vi "DC Motor Controller (FPGA).vi"() -> ()   [LabVIEW 2017]
doc: "Implements the FPGA controller of the Robotics Starter Kit motors.\n\nThis example is configured to run on a Single-board RIO 9631 and needs to be compiled. If you have a different RIO device, you must add the appropriate RIO targets to your LabVIEW Project and move the VIs in this project to the new target. You must also configure the IP address of the RIO target to match your network configuration."
uses:
  <vilib>/Platform/TimedLoop/XDataNode/timing_clust.ctl
  <vilib>/Platform/TimedLoop/XDataNode/nitl_modes.ctl
  <vilib>/Platform/TimedLoop/XDataNode/wakeup.ctl
  <vilib>/robotics/Utilities/Encoder Count Encoding.ctl
  <vilib>/rvi/Emulation/niFpgaSctlEmulationGetInTimedLoop.vi
  <vilib>/rvi/Emulation/niFpgaProcessEmulError.vi
  <vilib>/robotics/Utilities/FPGA Utilities/Count Two Phase Digital Encoder.vi
  <vilib>/rvi/eio/common/nirviEmuTemplateMethod_errors.vi
  <vilib>/rvi/Emulation/niFpgaGetClockAttributes.vi
  <vilib>/rvi/Emulation/niFpgaEmulationReportErrorSimple.vi
  Support VIs/DCMotor FPGA Globals.vi
  <vilib>/robotics/Utilities/FPGA Utilities/Generate Digital Pulse (uSec).vi
  <vilib>/rvi/Emulation/niFpgaCriticalErrorInLSC.vi
  <vilib>/eio/EIONode/EIONode.xnode
  <vilib>/addons/control/pid/fpga.llb/XNode/niFpgaPID.xnode
  <vilib>/Platform/TimedLoop/XDataNode/XDataNode.xnode
  <vilib>/robotics/Utilities/NI_Robotics Utilities.lvlib
  <vilib>/Platform/TimedLoop/XDataNode/XDNodeRunTimeDep.lvlib
  <vilib>/robotics/Utilities/FPGA Utilities/NI_Robotics_FPGA Utilities.lvlib
panel:
  in  "S 7":bool
  in  "Servo 7":u32(slide) scale=0.0..3000.0
  in  "invert pulse (F)":bool=TRUE
  in  "S6_timer":u16
  in  "S6_prev":u32
  in  "Indication":bool
  out "M1_finished":bool
  out "M0_finished":bool
  in  "DCmotor_1_B":bool
  in  "DCmotor_0_B":bool
  in  "M2_B":bool
  in  "Motor Power":u32(slide) scale=0.0..1000.0
  in  "M2_A":bool
  in  "Servo 4":u32(slide) scale=0.0..3000.0
  in  "Servo 5":u32(slide) scale=0.0..3000.0
  in  "Servo 6":u32(slide) scale=0.0..3000.0
  in  "S 4":bool
  in  "S 5":bool
  in  "S 6":bool
  in  "Slow velocity":i32=5
  in  "Ticks to slow":i32=360
  in  "Ticks to stop":i32=6
  in  "DCmotor_1_enc trgt":i32
  in  "DCmotor_0_enc trgt":i32
  in  "Left Encoder B":refnum<k21>="ConnectorB/DIO4"
  in  "Left Encoder A":refnum<k21>="ConnectorB/DIO3"
  in  "Right Encoder B":refnum<k21>="ConnectorA/DIO4"
  in  "Right Encoder A":refnum<k21>="ConnectorA/DIO3"
  in  "Right Motor":refnum<k21>="ConnectorB/DIO9"
  in  "Left Motor":refnum<k21>="ConnectorB/DIO8"
  in  "M0_B":refnum<k21>="ConnectorB/DIO6"
  in  "M0_A":refnum<k21>="ConnectorB/DIO5"
  in  "M1_B":refnum<k21>="ConnectorB/DIO7"
  in  "M1_A":refnum<k21>="ConnectorB/DIO13"
  out "DCmotor_0_enc":i32
  out "DCmotor_1_enc":i32
  in  "DCmotor_1_A":bool
  in  "DCmotor_0_A":bool
  in  "stop":bool
  in  "motor PID gains":T1={"proportional gain (Kc)"=2.5, "integral gain (Kc*Ts/Ti)"=0.01171875, "derivative gain (Kc*Td/Ts)"=0.01171875}
  in  "DCmotor_0_ccw vel sp":i32
  in  "DCmotor_1_ccw vel sp":i32
  out "DCmotor_0_ccw vel":i32
  out "DCmotor_1_ccw vel":i32
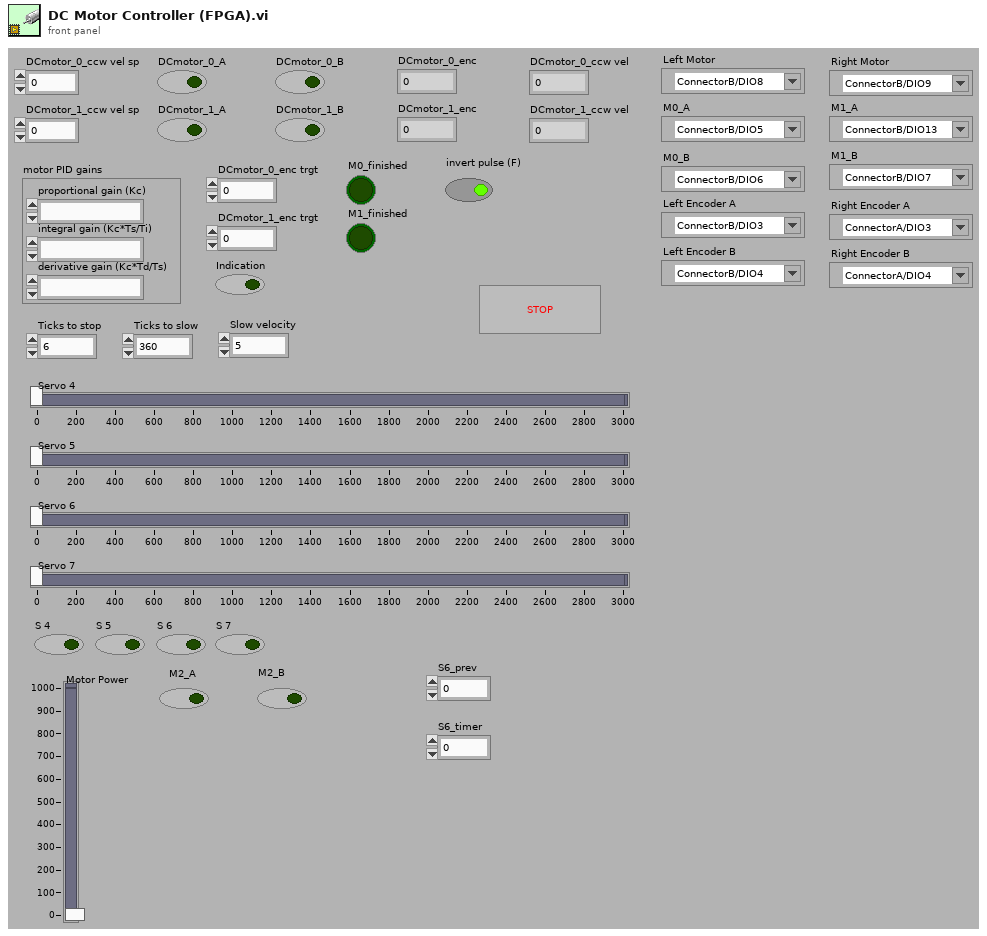
[diagram p1: front panel]
types:
  T1 = cluster{"proportional gain (Kc)":fxp<+/-,16,8>, "integral gain (Kc*Ts/Ti)":fxp<+/-,16,8>, "derivative gain (Kc*Td/Ts)":fxp<+/-,16,8>}
  T2 = cluster{"PID gains":cluster{"proportional gain (Kc)":fxp<+/-,16,8>, "integral gain (Kc*Ts/Ti)":fxp<+/-,16,8>, "derivative gain (Kc*Td/Ts)":fxp<+/-,16,8>}, "output range":cluster{"output high":fxp<+/-,16,16>, "output low":fxp<+/-,16,16>}, "setpoint":fxp<+/-,16,16>, "channel index":u16}
  T3 = cluster{"PID gains (x 2^8)":cluster{"proportional gain (Kc)":i16, "integral gain (Kc*Ts/Ti)":i16, "derivative gain (Kc*Td/Ts)":i16}, "output range":cluster{"output high":i16, "output low":i16}, "setpoint":i16, "channel index":u16}
  T4 = typedef "XDNodeRunTimeDep.lvlib/timing_clust.ctl" = cluster{"Expected End [f-1]":u64, "Actual End [f-1]":u64, "Finished Late? [f-1]":bool, "Expected End [i-1]":u64, "Actual End [i-1]":u64, "Finished Late? [i-1]":bool, "Expected Start [i]":u64, "Actual Start [i]":u64, "Expected Start [f]":u64, "Actual Start [f]":u64, "Source Name":string, "Structure Name":string, "Period":i64, "Deadline":i64, "Offset":i64, "Start":i64, "Priority":i32, "Timeout":i32, "Mode":T5, "Wakeup Reason":T6, "Error":errorcluster, "Source Type":string, "Secondary Source Type":string, "Global End Time":u64, "Global Start Time":u64, "Frame Duration":u64, "Iteration Duration":u64, "Assigned CPU":i32, "I/O Scan Engine Mode":u32}
  T5 = typedef "XDNodeRunTimeDep.lvlib/nitl_modes.ctl" = enum32{"No Change", "Process missed periods, maintain original phase", "Discard missed periods, maintain original phase", "Process missed periods, ignore original phase", "Discard missed periods, ignore original phase"}
  T6 = typedef "XDNodeRunTimeDep.lvlib/wakeup.ctl" = enum32{"Normal", "Aborted", "Asynchronous wakeup", "Timing source error", "Timed loop error", "Timeout"}
  T7 = typedef "NI_Robotics Utilities.lvlib/Encoder Count Encoding.ctl" = enum16{"X1", "X2", "X4"}
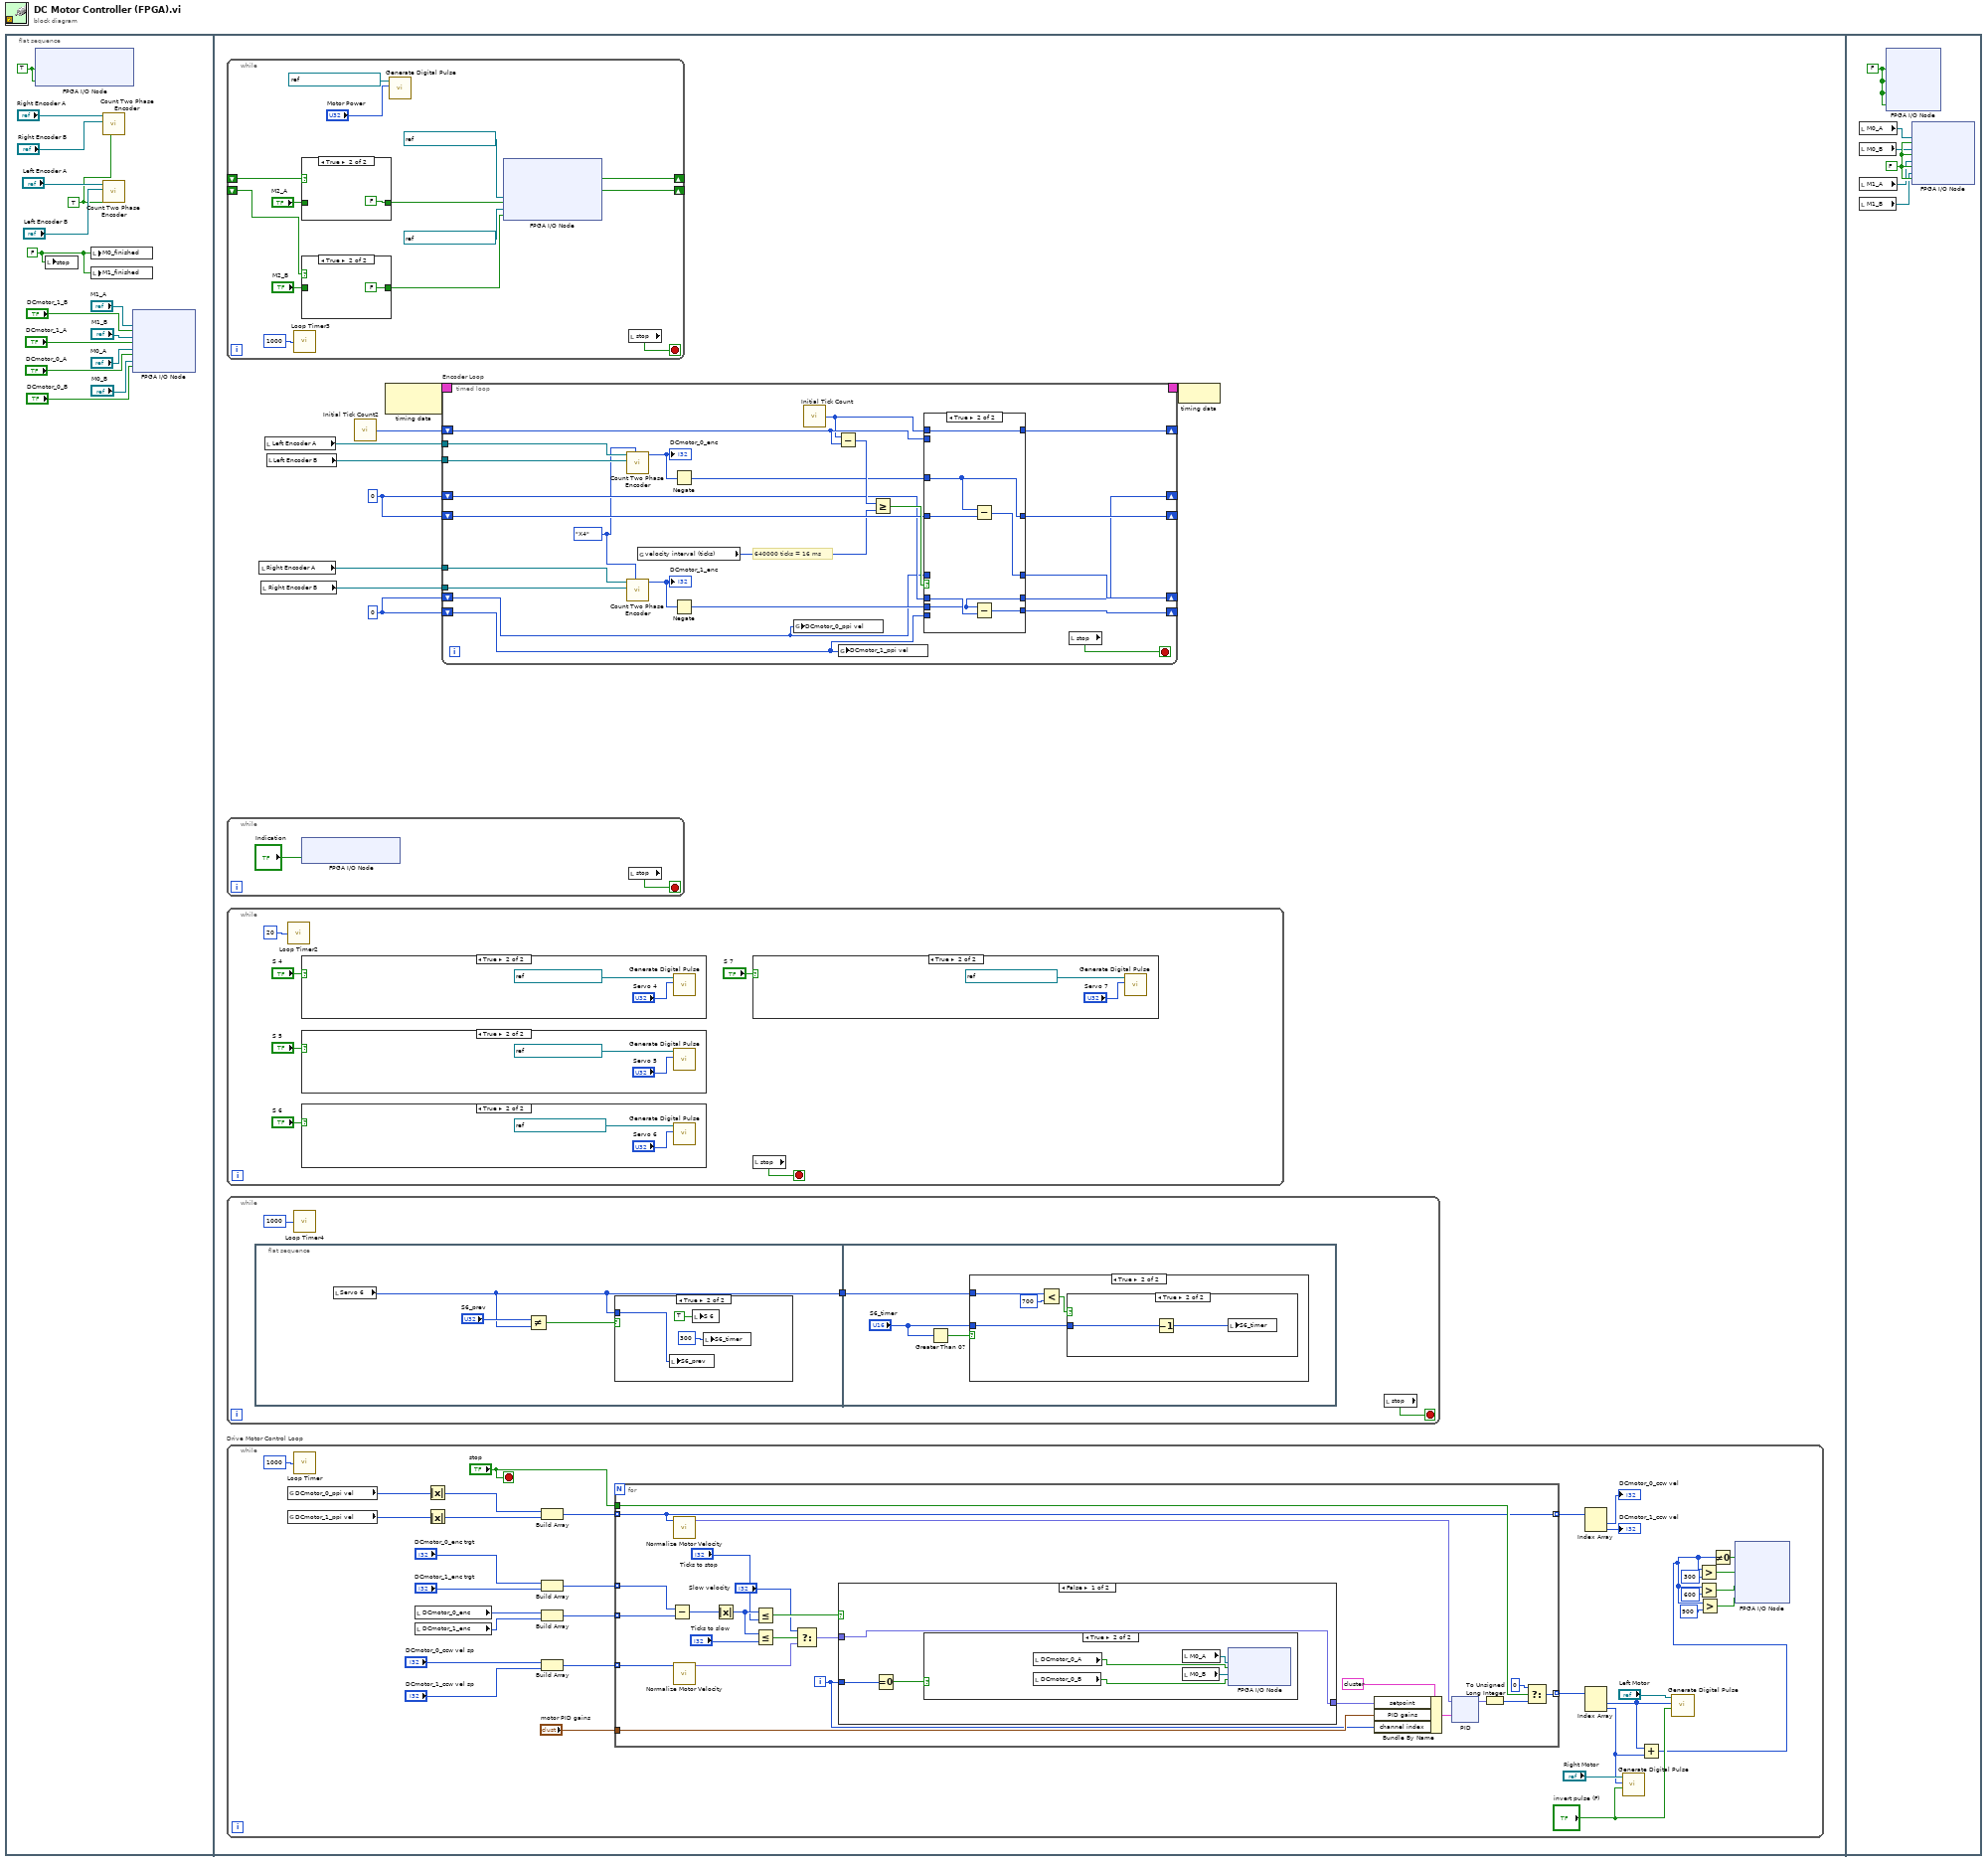
[diagram p0: block diagram]
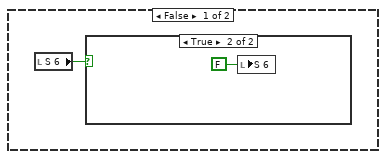
[diagram p3: hidden frame]
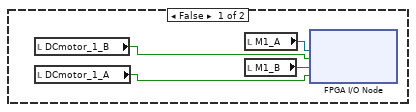
[diagram p12: hidden frame]
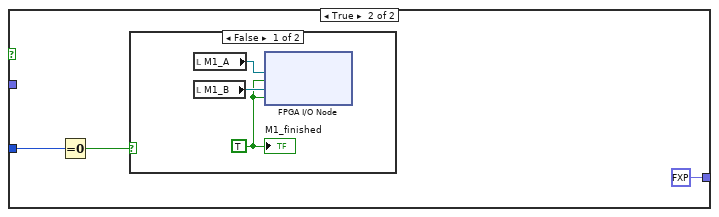
[diagram p13: hidden frame]
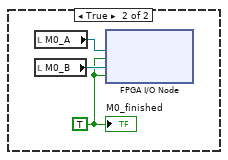
[diagram p14: hidden frame]
diagram:
  n1 = flat-sequence {
    frame #0 {
      w6 = TRUE ("ConnectorC/DIO0")
      w11 = TRUE ("reset (F)")
      w1 = FALSE ("stop")
      n2 = xnode "FPGA I/O Node"("ConnectorC/DIO2"=w6, "ConnectorC/DIO4"=w6) -> ()  [unwired: 2 in, 2 out]
      n3 = local write "stop"(w1) -> ()
      n4 = local write "M0_finished"(w1) -> ()
      n5 = local write "M1_finished"(w1) -> ()
      n6 = call-poly <vilib>:"Count Two Phase Encoder.vi"("reset (F)"=w11, "phase B FPGA digital input"="Right Encoder B", "phase A FPGA digital input"="Right Encoder A") -> ()  [unwired: 7 in, 2 out]
      n7 = call-poly <vilib>:"Count Two Phase Encoder.vi"("reset (F)"=w11, "phase B FPGA digital input"="Left Encoder B", "phase A FPGA digital input"="Left Encoder A") -> ()  [unwired: 7 in, 2 out]
      n8 = xnode "FPGA I/O Node"("I/O Item"="DCmotor_1_B", "FPGA I/O In"="M1_A", "I/O Item"="DCmotor_1_A", "FPGA I/O In"="M1_B", "I/O Item"="DCmotor_0_A", "FPGA I/O In"="M0_A", "I/O Item"="DCmotor_0_B", "FPGA I/O In"="M0_B") -> ()  [unwired: 4 out]
    }
    frame #1 {
      w20 = 0
      w21 = 0 ("Reset Position Value")
      n9 = while {
        shift-right: [w52] -> _
        shift-left: _ -> [w51]
        shift-right: [w50] -> _
        shift-left: _ -> [w49]
        stop <- w55 stop-if-true
        n10 = call "Loop Timer3"("Count(uSec)"=u32 1000) -> ()  [unwired: 1 out]
        n11 = case shown="True" w51 {
          tunnel: [w63 FALSE] -> w54
          tunnel: "M2_A" -> [w63 _]
          frame False {
          }
          frame True {
          }
        }
        n12 = case shown="True" w49 {
          tunnel: [w61 FALSE] -> w47
          tunnel: "M2_B" -> [w61 _]
          frame False {
          }
          frame True {
          }
        }
        n13 = call-poly <vilib>:"Generate Digital Pulse.vi"("pulse width (uSec)"="Motor Power", "FPGA digital output"=refnum<k21> "ConnectorA/DIO15") -> ()  [unwired: 10 in]
        n14 = xnode "FPGA I/O Node"("I/O Item"=w54, "FPGA I/O In"=refnum<k21> "ConnectorA/DIO14", "I/O Item"=w47, "FPGA I/O In"=refnum<k21> "ConnectorA/DIO13") -> ("ConnectorC/DIO1"=w52:bool, "ConnectorC/DIO3"=w50:bool)  [unwired: 2 in, 4 out]
        n15 = local read "stop"() -> (w55:bool)
      }
      n16 = while {
        stop <- w45 stop-if-true
        n17 = xnode "FPGA I/O Node"("ConnectorC/DIO0"="Indication") -> ()  [unwired: 1 in, 1 out]
        n18 = local read "stop"() -> (w45:bool)
      }
      n19 = while {
        stop <- w66 stop-if-true
        n20 = call "Loop Timer2"("Count(mSec)"=u32 20) -> ()  [unwired: 1 out]
        n21 = case shown="True" "S 4" {
          frame False {
          }
          frame True {
            n22 = call-poly <vilib>:"Generate Digital Pulse.vi"("pulse width (uSec)"="Servo 4", "FPGA digital output"=refnum<k21> "ConnectorA/DIO8") -> ()  [unwired: 10 in]
          }
        }
        n23 = case shown="True" "S 5" {
          frame False {
          }
          frame True {
            n24 = call-poly <vilib>:"Generate Digital Pulse.vi"("pulse width (uSec)"="Servo 5", "FPGA digital output"=refnum<k21> "ConnectorA/DIO9") -> ()  [unwired: 10 in]
          }
        }
        n25 = case shown="True" "S 6" {
          frame False {
          }
          frame True {
            n26 = call-poly <vilib>:"Generate Digital Pulse.vi"("pulse width (uSec)"="Servo 6", "FPGA digital output"=refnum<k21> "ConnectorA/DIO10") -> ()  [unwired: 10 in]
          }
        }
        n27 = local read "stop"() -> (w66:bool)
        n28 = case shown="True" "S 7" {
          frame False {
          }
          frame True {
            n29 = call-poly <vilib>:"Generate Digital Pulse.vi"("pulse width (uSec)"="Servo 7", "FPGA digital output"=refnum<k21> "ConnectorB/DIO10") -> ()  [unwired: 10 in]
          }
        }
      }
      n30 = while {
        stop <- w27 stop-if-true
        n31 = flat-sequence {
          tunnel: [w28] -> w25
          tunnel: w25 -> [w34]
          frame #0 {
            n32 = local read "Servo 6"() -> (w28:u32)
            n33 = Not Equal?(x="S6_prev", y=w28) -> (x != y?=w29:bool)
            n34 = case shown="True" w29 {
              tunnel: w28 -> [_ w31]
              frame False {
              }
              frame True {
                n35 = local write "S6_prev"(w31) -> ()
                n36 = local write "S 6"(TRUE ("S 6")) -> ()
                n37 = local write "S6_timer"(u16 300 ("S6_timer")) -> ()
              }
            }
          }
          frame #1 {
            n38 = Greater Than 0?(x="S6_timer") -> (x > 0?=w35:bool)
            n39 = case shown="True" w35 {
              tunnel: "S6_timer" -> [_ w42]
              tunnel: w34 -> [_ w41]
              frame False {
                n40 = local read "S 6"() -> (w37:bool)
                n41 = case shown="True" w37 {
                  frame False {
                  }
                  frame True {
                    n42 = local write "S 6"(FALSE ("S 6")) -> ()
                  }
                }
              }
              frame True {
                n43 = Less?(x=w41, y=u32 700) -> (x < y?=w39:bool)
                n44 = case shown="True" w39 {
                  tunnel: w42 -> [_ w43]
                  frame False {
                  }
                  frame True {
                    n45 = Decrement(x=w43) -> (x-1=w44:u16)
                    n46 = local write "S6_timer"(w44) -> ()
                  }
                }
              }
            }
          }
        }
        n47 = call "Loop Timer4"("Count(uSec)"=u32 1000) -> ()  [unwired: 1 out]
        n48 = local read "stop"() -> (w27:bool)
      }
      n49 = while "Drive Motor Control Loop" {
        stop <- "stop" stop-if-true
        n50 = global read "DCMotor FPGA Globals.vi" "DCmotor_0_ppi vel"() -> (w106:i32)
        n51 = global read "DCMotor FPGA Globals.vi" "DCmotor_1_ppi vel"() -> (w105:i32)
        n52 = call "Loop Timer"("Count(uSec)"=u32 1000) -> ()  [unwired: 1 out]
        n53 = local read "DCmotor_0_enc"() -> (w94:i32)
        n54 = local read "DCmotor_1_enc"() -> (w93:i32)
        n55 = Absolute Value(x=w106) -> (abs(x)=w107:i32)
        n56 = Absolute Value(x=w105) -> (abs(x)=w104:i32)
        n57 = Build Array(w107, w104) -> (w111:i32[])
        n58 = Build Array("DCmotor_0_enc trgt", "DCmotor_1_enc trgt") -> (w95:i32[])
        n59 = Build Array(w94, w93) -> (w92:i32[])
        n60 = Build Array("DCmotor_0_ccw vel sp", "DCmotor_1_ccw vel sp") -> (w110:i32[])
        n61 = for {
          tunnel: "motor PID gains" -> [w134]
          tunnel: w111 -> [w113] mode=indexing
          tunnel: [w113] -> w109 mode=indexing
          tunnel: w110 -> [w133] mode=indexing
          tunnel: [w128] -> w108 mode=indexing
          tunnel: "stop" -> [w131]
          tunnel: w95 -> [w127] mode=indexing
          tunnel: w92 -> [w126] mode=indexing
          i -> [w118]
          n62 = Subtract(x=w127, y=w126) -> (x-y=w125:i32)
          n63 = call "Normalize Motor Velocity.vi"("velocity (rad/s)"=w113) -> ("normalized velocity"=w114:fxp<+/-,16,16>)  [unwired: 10 in]
          n64 = call "Normalize Motor Velocity.vi"("velocity (rad/s)"=w133) -> ("normalized velocity"=w123:fxp<+/-,16,16>)  [unwired: 10 in]
          n65 = Absolute Value(x=w125) -> (abs(x)=w122:i32)
          n66 = Less Or Equal?(x=w122, y="Ticks to stop") -> (x <= y?=w121:bool)
          n67 = Less Or Equal?(x=w122, y="Ticks to slow") -> (x <= y?=w124:bool)
          n68 = Select(t="Slow velocity", s=w124, f=w123) -> (s? t:f=w119:fxp<+/-,32,32>)
          n69 = case shown="False" w121 {
            tunnel: [w139 fxp<+/-,16,16> -1.0 ("normalized velocity")] -> w120
            tunnel: w119 -> [w139 _]
            tunnel: w118 -> [w137 w148]
            frame False {
              n70 = Equal To 0?(x=w137) -> (x = 0?=w138:bool)
              n71 = case shown="True" w138 {
                frame False {
                  n72 = local read "DCmotor_1_B"() -> (w141:bool)
                  n73 = local read "DCmotor_1_A"() -> (w140:bool)
                  n74 = local read "M1_A"() -> (w143:refnum<k21>)
                  n75 = local read "M1_B"() -> (w142:refnum<k21>)
                  n76 = xnode "FPGA I/O Node"("I/O Item"=w141, "FPGA I/O In"=w143, "I/O Item"=w140, "FPGA I/O In"=w142) -> ()  [unwired: 2 out]
                }
                frame True {
                  n77 = local read "DCmotor_0_A"() -> (w145:bool)
                  n78 = local read "DCmotor_0_B"() -> (w144:bool)
                  n79 = local read "M0_A"() -> (w147:refnum<k21>)
                  n80 = local read "M0_B"() -> (w146:refnum<k21>)
                  n81 = xnode "FPGA I/O Node"("I/O Item"=w145, "FPGA I/O In"=w147, "I/O Item"=w144, "FPGA I/O In"=w146) -> ()  [unwired: 2 out]
                }
              }
            }
            frame True {
              n82 = Equal To 0?(x=w148) -> (x = 0?=w149:bool)
              n83 = case shown="False" w149 {
                frame False {
                  w151 = TRUE
                  n84 = local read "M1_A"() -> (w153:refnum<k21>)
                  n85 = local read "M1_B"() -> (w152:refnum<k21>)
                  n86 = xnode "FPGA I/O Node"("I/O Item"=w151, "FPGA I/O In"=w153, "I/O Item"=w151, "FPGA I/O In"=w152) -> ()  [unwired: 2 out]
                  "M1_finished" <- w151
                }
                frame True {
                  w154 = TRUE
                  n87 = local read "M0_A"() -> (w156:refnum<k21>)
                  n88 = local read "M0_B"() -> (w155:refnum<k21>)
                  n89 = xnode "FPGA I/O Node"("I/O Item"=w154, "FPGA I/O In"=w156, "I/O Item"=w154, "FPGA I/O In"=w155) -> ()  [unwired: 2 out]
                  "M0_finished" <- w154
                }
              }
            }
          }
          n90 = Bundle By Name(cluster=T2 {"PID gains"={"proportional gain (Kc)"=0.00390625, "integral gain (Kc*Ts/Ti)"=0.00390625, "derivative gain (Kc*Td/Ts)"=0.00390625}, "output range"={"output high"=1000.0, "output low"=0.0}, "setpoint"=0.0, "channel index"=0} ("configuration"), "setpoint"=w120, "PID gains"=w134, "channel index"=w118) -> (w135:T2)
          n91 = xnode ("PID")("process variable"=w114, "configuration"=w135) -> ("output"=w132:fxp<+/-,16,16>)  [unwired: 1 in, 1 out]
          n92 = To Unsigned Long Integer(number=w132) -> (unsigned 32bit integer=w130:u32)
          n93 = Select(t=u32 0, s=w131, f=w130) -> (s? t:f=w128:u32)
        }
        n94 = Index Array(array=w109) -> (element #1=→"DCmotor_0_ccw vel":i32, element #2=→"DCmotor_1_ccw vel":i32)  [unwired: 2 in]
        n95 = Index Array(array=w108) -> (element #1=w88:u32, element #2=w87:u32)  [unwired: 2 in]
        n96 = call-poly <vilib>:"Generate Digital Pulse.vi"("invert pulse (F)"="invert pulse (F)", "pulse width (uSec)"=w87, "FPGA digital output"="Right Motor") -> ()  [unwired: 9 in]
        n97 = Add(x=w88, y=w87) -> (x+y=w86:u32)
        n98 = call-poly <vilib>:"Generate Digital Pulse.vi"("invert pulse (F)"="invert pulse (F)", "pulse width (uSec)"=w88, "FPGA digital output"="Left Motor") -> ()  [unwired: 9 in]
        n99 = Greater?(x=w86, y=u32 300) -> (0:w84:bool)
        n100 = Greater?(x=w86, y=u32 600) -> (0:w82:bool)
        n101 = Greater?(x=w86, y=u32 900) -> (0:w80:bool)
        n102 = Not Equal To 0?(x=w86) -> (x != 0?=w85:bool)
        n103 = xnode "FPGA I/O Node"("LED0"=w85, "LED1"=w84, "LED2"=w82, "LED3"=w80) -> ()  [unwired: 4 in, 4 out]
      }
      n104 = local read "Right Encoder A"() -> (w17:refnum<k21>)
      n105 = local read "Right Encoder B"() -> (w16:refnum<k21>)
      n106 = local read "Left Encoder A"() -> (w19:refnum<k21>)
      n107 = local read "Left Encoder B"() -> (w18:refnum<k21>)
      n108 = call "Initial Tick Count2"() -> ("Tick Count(Ticks)"=w22:u32)
      n109 = node-c288() -> (w24:T4)  [unwired: 1 in]
      n110 = timed-loop "Encoder Loop" {
        timing: w24 -> [_]
        timing-out: [_] -> w23
        shift-right: [w200] -> _
        shift-left: w22 -> [w205]
        shift-right: [w201] -> _
        shift-left: w21 -> [w203]
        shift-right: [w202] -> _
        shift-left: w20 -> [w191]
        shift-right: [w198] -> _
        shift-left: w21 -> [w199]
        shift-right: [w197] -> _
        shift-left: w20 -> [w190]
        tunnel: w19 -> [w194]
        tunnel: w18 -> [w193]
        tunnel: w17 -> [w184]
        tunnel: w16 -> [w185]
        stop <- w186 stop-if-true
        w192 = Encoder_Count_Encoding."X4" ("count multiplier (X1)")
        # "640000 ticks = 16 ms"
        n111 = call-poly <vilib>:"Count Two Phase Encoder.vi"("count encoding (X1)"=w192, "phase B FPGA digital input"=w193, "phase A FPGA digital input"=w194) -> ("new count"=w187:i32)  [unwired: 7 in, 1 out]
        "DCmotor_0_enc" <- w187
        n112 = call-poly <vilib>:"Count Two Phase Encoder.vi"("count encoding (X1)"=w192, "phase B FPGA digital input"=w185, "phase A FPGA digital input"=w184) -> ("new count"=w188:i32)  [unwired: 7 in, 1 out]
        "DCmotor_1_enc" <- w188
        n113 = global read "DCMotor FPGA Globals.vi" "velocity interval (ticks)"() -> (w189:u32)
        n114 = Negate(x=w187) -> (-x=w196:i32)
        n115 = Negate(x=w188) -> (-x=w195:i32)
        n116 = global write "DCMotor FPGA Globals.vi" "DCmotor_0_ppi vel"(w191) -> ()
        n117 = call "Initial Tick Count"() -> ("Tick Count(Ticks)"=w204:u32)
        n118 = Subtract(x=w204, y=w205) -> (x-y=w207:u32)
        n119 = global write "DCMotor FPGA Globals.vi" "DCmotor_1_ppi vel"(w190) -> ()
        n120 = Greater Or Equal?(x=w207, y=w189) -> (x >= y?=w206:bool)
        n121 = case shown="True" w206 {
          tunnel: w204 -> [_ w218]
          tunnel: w205 -> [w212 _]
          tunnel: [w212 w218] -> w200
          tunnel: w203 -> [w211 w219]
          tunnel: [w211 w217] -> w201
          tunnel: w196 -> [_ w217]
          tunnel: [w210 w216] -> w202
          tunnel: w191 -> [w210 _]
          tunnel: w199 -> [w209 w215]
          tunnel: w190 -> [w208 _]
          tunnel: [w209 w214] -> w198
          tunnel: [w208 w213] -> w197
          tunnel: w195 -> [_ w214]
          frame False {
          }
          frame True {
            n122 = Subtract(x=w217, y=w219) -> (x-y=w216:i32)
            n123 = Subtract(x=w214, y=w215) -> (x-y=w213:i32)
          }
        }
        n124 = local read "stop"() -> (w186:bool)
      }
      n125 = node-c288(w23) -> ()
    }
    frame #2 {
      w224 = FALSE
      w229 = FALSE
      n126 = local read "M0_A"() -> (w225:refnum<k21>)
      n127 = local read "M0_B"() -> (w226:refnum<k21>)
      n128 = local read "M1_A"() -> (w227:refnum<k21>)
      n129 = local read "M1_B"() -> (w228:refnum<k21>)
      n130 = xnode "FPGA I/O Node"("LED0"=w224, "LED1"=w224, "LED2"=w224, "LED3"=w224) -> ()  [unwired: 4 in, 4 out]
      n131 = xnode "FPGA I/O Node"("I/O Item"=w229, "FPGA I/O In"=w225, "I/O Item"=w229, "FPGA I/O In"=w226, "I/O Item"=w229, "FPGA I/O In"=w227, "I/O Item"=w229, "FPGA I/O In"=w228) -> ()  [unwired: 4 out]
    }
  }
